vi "Get Map Collection Data Size.vi"(8 "error in (no error)":errorcluster, 10 "Data String":u8[](array[numeric]), 11 "Type Descriptor":i16[](array[numeric])) -> (0 "error out":errorcluster, 2 "Data Size":i32)   [LabVIEW 2017, in "Composition.lvlib"]
doc: "Gets the data size of a map collection."
uses:
  Composition.lvlib
  Get Data Type.vi/2a0888ac-0230-421b-a610-ddb651202d87.vi
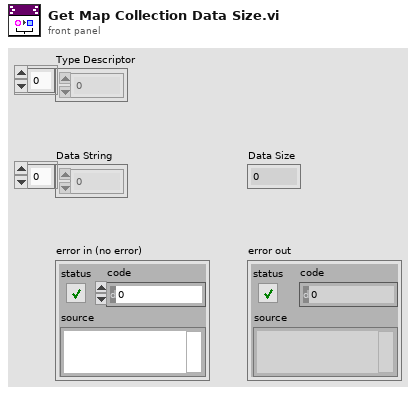
[diagram p1: front panel]
types:
  T1 = typedef "Composition.lvlib/Data Type.ctl" = enum16{"Void", "I8", "I16", "I32", "I64", "U8", "U16", "U32", "U64", "SGL", "DBL", "EXT", "CSG", "CDB", "CXT", "0x0F", "0x10", "0x11", "0x12", "0x13", "0x14", "Enum U8", "Enum U16", "Enum U32", "0x18", "SGL Physical", "DBL Physical", "EXT Physical", "CSG Physical", "CDB Physical", "CXT Physical", "0x1F", "Boolean U16", "Boolean U8", "0x22", "0x23", "0x24", "0x25", "0x26", "0x27", "0x28", "0x29", "0x2A", "0x2B", "0x2C", "0x2D", "0x2E", "0x2F", "String", "0x31", "Path", "Picture", "CString", "PString", "0x36", "Tag", "0x38", "0x39", "0x3A", "0x3B", "0x3C", "0x3D", "0x3E", "SubString", "Array", "Array Data Ptr", "0x42", "0x43", "0x44", "0x45", "0x46", "0x47", "0x48", "0x49", "0x4A", "0x4B", "0x4C", "0x4D", "0x4E", "SubArray", "Cluster", "0x51", "0x52", "Variant", "Waveform", "0x55", "0x56", "0x57", "0x58", "0x59", "0x5A", "0x5B", "0x5C", "0x5D", "CFX", "FXP", "Block", "Type Block", "Void Block", "Aligned Block", "Repeated Block", "Alignment Marker", "0x66", "0x67", "0x68", "0x69", "0x6A", "0x6B", "0x6C", "0x6D", "0x6E", "0x6F", "Refnum", "0x71", "0x72", "Set Collection", "Map Collection", "0x75", "0x76", "0x77", "0x78", "0x79", "0x7A", "0x7B", "0x7C", "0x7D", "0x7E", "0x7F", "Ptr", "0x81", "0x82", "Ptr to", "EXT Data", "0x85", "0x86", "0x87", "0x88", "0x89", "0x8A", "0x8B", "0x8C", "0x8D", "0x8E", "0x8F", "0x90", "0x91", "0x92", "0x93", "0x94", "0x95", "0x96", "0x97", "0x98", "0x99", "0x9A", "0x9B", "0x9C", "0x9D", "0x9E", "0x9F", "Array Interface", "Interface to Data", "0xA2", "0xA3", "0xA4", "0xA5", "0xA6", "0xA7", "0xA8", "0xA9", "0xAA", "0xAB", "0xAC", "0xAD", "0xAE", "0xAF", "0xB0", "0xB1", "0xB2", "0xB3", "0xB4", "0xB5", "0xB6", "0xB7", "0xB8", "0xB9", "0xBA", "0xBB", "0xBC", "0xBD", "0xBE", "0xBF", "0xC0", "0xC1", "0xC2", "0xC3", "0xC4", "0xC5", "0xC6", "0xC7", "0xC8", "0xC9", "0xCA", "0xCB", "0xCC", "0xCD", "0xCE", "0xCF", "0xD0", "0xD1", "0xD2", "0xD3", "0xD4", "0xD5", "0xD6", "0xD7", "0xD8", "0xD9", "0xDA", "0xDB", "0xDC", "0xDD", "0xDE", "0xDF", "0xE0", "0xE1", "0xE2", "0xE3", "0xE4", "0xE5", "0xE6", "0xE7", "0xE8", "0xE9", "0xEA", "0xEB", "0xEC", "0xED", "0xEE", "0xEF", "Function", "TypeDef", "PolyVI", "0xF3", "0xF4", "0xF5", "0xF6", "0xF7", "0xF8", "0xF9", "0xFA", "0xFB", "0xFC", "0xFD", "0xFE", "0xFF"}
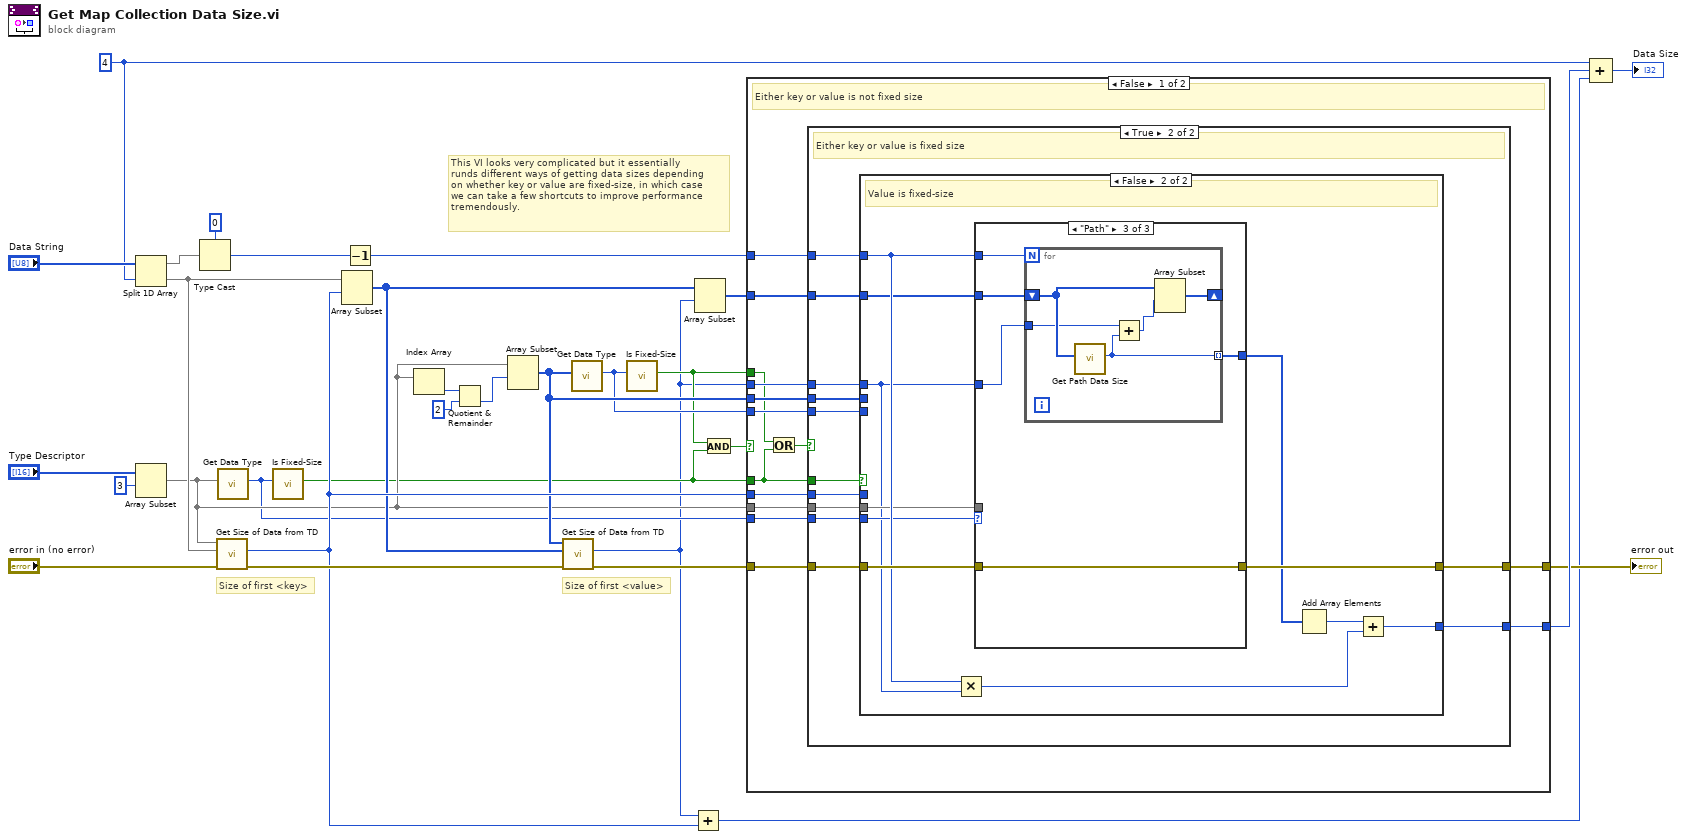
[diagram p0: block diagram]
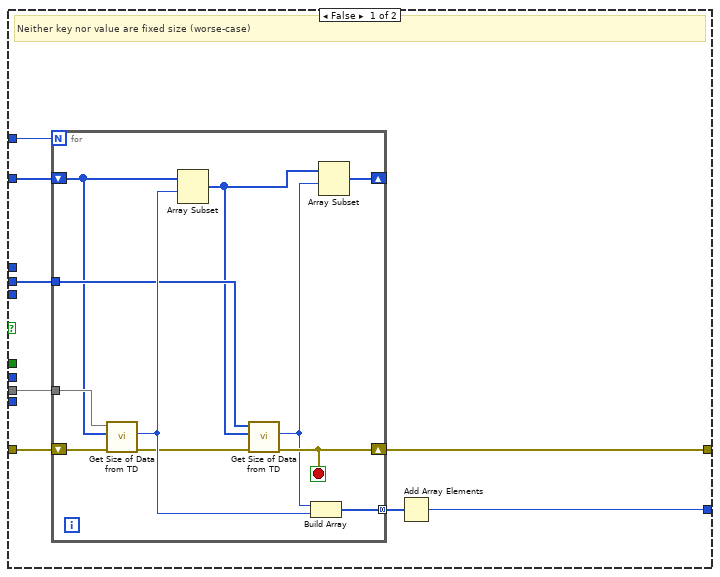
[diagram p2: hidden frame]
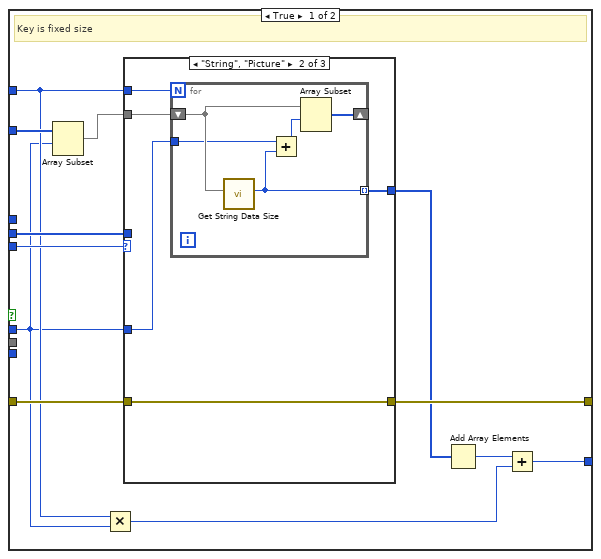
[diagram p3: hidden frame]
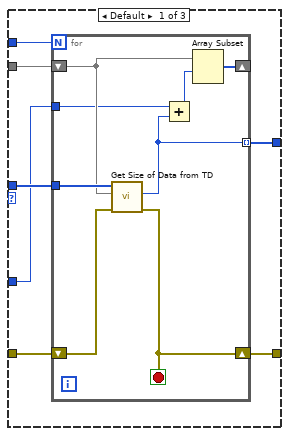
[diagram p4: hidden frame]
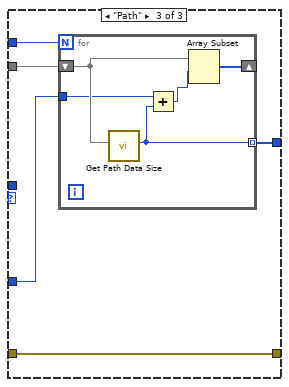
[diagram p5: hidden frame]
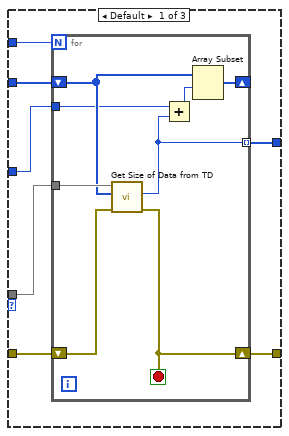
[diagram p6: hidden frame]
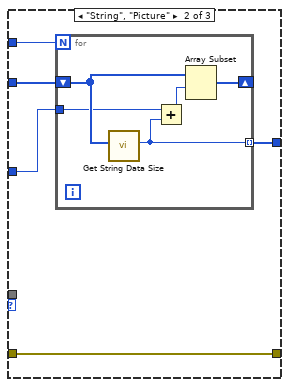
[diagram p7: hidden frame]
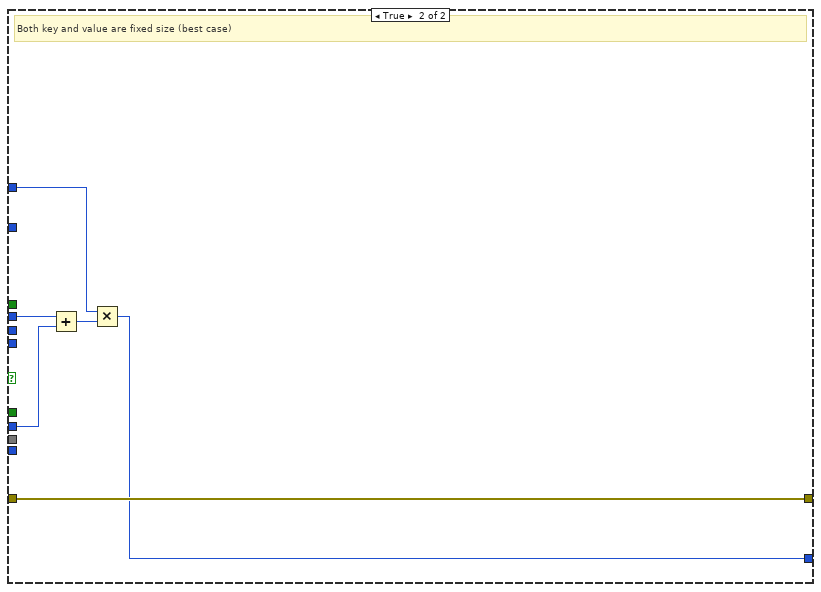
[diagram p8: hidden frame]
diagram:
  w10 = 4 ("index")
  # "This VI looks very complicated but it essentially\nrunds different ways of getting data sizes depending\non whether key or value are fixed-size, in which case\nwe can take a few shortcuts to improve performance\ntremendously."
  # "Size of first <value>"
  # "Size of first <key>"
  n1 = Split 1D Array(array="Data String", index=w10) -> (first subarray=w28:u8[], second subarray=w17:u8[])
  n2 = Array Subset(array="Type Descriptor", index=3) -> (w6:i16[])  [unwired: 1 in]
  n3 = Type Cast(type=0, x=w28) -> (*(type *) &x=w27:i32)
  n4 = call "Get Size of Data from TD.vi"("error in (no error)"="error in (no error)", "Data String"=w17, "Type Descriptor"=w6) -> ("error out"=w16:errorcluster, "Size of Data"=w14:i32)  [unwired: 7 in]
  n5 = call "Get Data Type.vi"("Type Descriptor"=w6) -> ("Data Type"=w5:T1)  [unwired: 10 in]
  n6 = call "Is Fixed-Size.vi"("Data Type"=w5) -> ("Is Fixed-Size"=w2:bool)  [unwired: 10 in]
  n7 = Array Subset(array=w17, index=w14) -> (w9:u8[])  [unwired: 1 in]
  n8 = Decrement(x=w27) -> (x-1=w15:i32)
  n9 = Index Array(array=w6) -> (element=w19:i16)  [unwired: 1 in]
  n10 = Quotient & Remainder(x=w19, y=i16 2) -> (floor(x/y)=w21:i16)  [unwired: 1 out]
  n11 = Array Subset(array=w6, index=w21) -> (w12:i16[])  [unwired: 1 in]
  n12 = call "Get Size of Data from TD.vi"("error in (no error)"=w16, "Data String"=w9, "Type Descriptor"=w12) -> ("error out"=w11:errorcluster, "Size of Data"=w1:i32)  [unwired: 7 in]
  n13 = call "Get Data Type.vi"("Type Descriptor"=w12) -> ("Data Type"=w7:T1)  [unwired: 10 in]
  n14 = call "Is Fixed-Size.vi"("Data Type"=w7) -> ("Is Fixed-Size"=w3:bool)  [unwired: 10 in]
  n15 = Add(x=w1, y=w14) -> (x+y=w13:i32)
  n16 = Array Subset(array=w9, index=w1) -> (w8:u8[])  [unwired: 1 in]
  n17 = And(x=w3, y=w2) -> (x .and. y?=w4:bool)
  n18 = case shown="False" w4 {
    tunnel: [w44 w169] -> w26
    tunnel: [w43 w174] -> w23
    tunnel: w15 -> [w42 w170]
    tunnel: w2 -> [w33 _]
    tunnel: w3 -> [w32 _]
    tunnel: w14 -> [w41 w172]
    tunnel: w12 -> [w40 _]
    tunnel: w11 -> [w39 w174]
    tunnel: w8 -> [w38 _]
    tunnel: w1 -> [w37 w173]
    tunnel: w7 -> [w36 _]
    tunnel: w6 -> [w35 _]
    tunnel: w5 -> [w34 _]
    frame False {
      # "Either key or value is not fixed size"
      n19 = Or(x=w32, y=w33) -> (x .or. y?=w31:bool)
      n20 = case shown="True" w31 {
        tunnel: [w51 w67] -> w44
        tunnel: [w50 w75] -> w43
        tunnel: w42 -> [w49 w74]
        tunnel: w33 -> [_ w69]
        tunnel: w41 -> [_ w68]
        tunnel: w40 -> [w48 w73]
        tunnel: w39 -> [w47 w72]
        tunnel: w38 -> [w46 w71]
        tunnel: w37 -> [_ w66]
        tunnel: w36 -> [_ w65]
        tunnel: w35 -> [w45 w70]
        tunnel: w34 -> [_ w64]
        frame False {
          # "Neither key nor value are fixed size (worse-case)"
          n21 = for {
            N: w49 -> [_]
            shift-right: [w63] -> _
            shift-left: w46 -> [w53]
            tunnel: [w61] -> w52 mode=concatenating
            shift-right: [w59] -> w50
            shift-left: w47 -> [w60]
            tunnel: w45 -> [w56]
            tunnel: w48 -> [w55]
            stop <- w59 stop-if-true
            n22 = call "Get Size of Data from TD.vi"("error in (no error)"=w60, "Data String"=w53, "Type Descriptor"=w56) -> ("error out"=w57:errorcluster, "Size of Data"=w62:i32)  [unwired: 7 in]
            n23 = Array Subset(array=w53, index=w62) -> (w54:u8[])  [unwired: 1 in]
            n24 = call "Get Size of Data from TD.vi"("error in (no error)"=w57, "Data String"=w54, "Type Descriptor"=w55) -> ("error out"=w59:errorcluster, "Size of Data"=w58:i32)  [unwired: 7 in]
            n25 = Build Array(w58, w62) -> (w61:i32[])
            n26 = Array Subset(array=w54, index=w58) -> (w63:u8[])  [unwired: 1 in]
          }
          n27 = Add Array Elements(numeric array=w52) -> (sum=w51:i32)
        }
        frame True {
          # "Either key or value is fixed size"
          n28 = case shown="False" w69 {
            tunnel: [w85 w132] -> w67
            tunnel: [w83 w130] -> w75
            tunnel: w74 -> [w79 w128]
            tunnel: w73 -> [w81 _]
            tunnel: w72 -> [w82 w129]
            tunnel: w71 -> [w87 w123]
            tunnel: w70 -> [_ w126]
            tunnel: w68 -> [w76 _]
            tunnel: w66 -> [_ w124]
            tunnel: w65 -> [w80 _]
            tunnel: w64 -> [_ w125]
            frame True {
              # "Key is fixed size"
              n29 = Array Subset(array=w87, index=w76) -> (w78:u8[])  [unwired: 1 in]
              n30 = Multiply(x=w79, y=w76) -> (x*y=w84:i32)
              n31 = case shown="\"String\", \"Picture\"" w80 {
                tunnel: w78 -> [w94 w106 w116]
                tunnel: w79 -> [w93 w107 w117]
                tunnel: [w89 w104 w114] -> w77
                tunnel: w81 -> [w92 _ _]
                tunnel: w82 -> [w91 w105 w115]
                tunnel: [w90 w105 w115] -> w83
                tunnel: w76 -> [w88 w103 w113]
                frame Default {
                  n32 = for {
                    N: w93 -> [_]
                    tunnel: w92 -> [w102]
                    shift-right: [w100] -> _
                    shift-left: w94 -> [w101]
                    tunnel: [w97] -> w89 mode=indexing
                    shift-right: [w98] -> w90
                    shift-left: w91 -> [w99]
                    tunnel: w88 -> [w96]
                    stop <- w98 stop-if-true
                    n33 = call "Get Size of Data from TD.vi"("error in (no error)"=w99, "Data String"=w101, "Type Descriptor"=w102) -> ("error out"=w98:errorcluster, "Size of Data"=w97:i32)  [unwired: 7 in]
                    n34 = Add(x=w96, y=w97) -> (x+y=w95:i32)
                    n35 = Array Subset(array=w101, index=w95) -> (w100:u8[])  [unwired: 1 in]
                  }
                }
                frame "String", "Picture" {
                  n36 = for {
                    N: w107 -> [_]
                    shift-right: [w112] -> _
                    shift-left: w106 -> [w111]
                    tunnel: [w110] -> w104 mode=indexing
                    tunnel: w103 -> [w108]
                    n37 = call "Get String Data Size.vi"("Data String"=w111) -> ("Data Size"=w110:i32)  [unwired: 10 in]
                    n38 = Add(x=w108, y=w110) -> (x+y=w109:i32)
                    n39 = Array Subset(array=w111, index=w109) -> (w112:u8[])  [unwired: 1 in]
                  }
                }
                frame "Path" {
                  n40 = for {
                    N: w117 -> [_]
                    shift-right: [w122] -> _
                    shift-left: w116 -> [w121]
                    tunnel: [w120] -> w114 mode=indexing
                    tunnel: w113 -> [w118]
                    n41 = call "Get Path Data Size.vi"("Data String"=w121) -> ("Data Size"=w120:i32)  [unwired: 10 in]
                    n42 = Add(x=w118, y=w120) -> (x+y=w119:i32)
                    n43 = Array Subset(array=w121, index=w119) -> (w122:u8[])  [unwired: 1 in]
                  }
                }
              }
              n44 = Add Array Elements(numeric array=w77) -> (sum=w86:i32)
              n45 = Add(x=w86, y=w84) -> (x+y=w85:i32)
            }
            frame False {
              # "Value is fixed-size"
              n46 = Multiply(x=w128, y=w124) -> (x*y=w131:i32)
              n47 = case shown="\"Path\"" w125 {
                tunnel: w123 -> [w140 w152 w162]
                tunnel: w128 -> [w139 w153 w163]
                tunnel: [w135 w150 w160] -> w127
                tunnel: w126 -> [w138 _ _]
                tunnel: w129 -> [w137 w151 w161]
                tunnel: [w136 w151 w161] -> w130
                tunnel: w124 -> [w134 w149 w159]
                frame Default {
                  n48 = for {
                    N: w139 -> [_]
                    tunnel: w138 -> [w148]
                    shift-right: [w146] -> _
                    shift-left: w140 -> [w147]
                    tunnel: [w143] -> w135 mode=indexing
                    shift-right: [w144] -> w136
                    shift-left: w137 -> [w145]
                    tunnel: w134 -> [w142]
                    stop <- w144 stop-if-true
                    n49 = call "Get Size of Data from TD.vi"("error in (no error)"=w145, "Data String"=w147, "Type Descriptor"=w148) -> ("error out"=w144:errorcluster, "Size of Data"=w143:i32)  [unwired: 7 in]
                    n50 = Add(x=w142, y=w143) -> (x+y=w141:i32)
                    n51 = Array Subset(array=w147, index=w141) -> (w146:u8[])  [unwired: 1 in]
                  }
                }
                frame "String", "Picture" {
                  n52 = for {
                    N: w153 -> [_]
                    shift-right: [w158] -> _
                    shift-left: w152 -> [w157]
                    tunnel: [w156] -> w150 mode=indexing
                    tunnel: w149 -> [w154]
                    n53 = call "Get String Data Size.vi"("Data String"=w157) -> ("Data Size"=w156:i32)  [unwired: 10 in]
                    n54 = Add(x=w154, y=w156) -> (x+y=w155:i32)
                    n55 = Array Subset(array=w157, index=w155) -> (w158:u8[])  [unwired: 1 in]
                  }
                }
                frame "Path" {
                  n56 = for {
                    N: w163 -> [_]
                    shift-right: [w168] -> _
                    shift-left: w162 -> [w167]
                    tunnel: [w166] -> w160 mode=indexing
                    tunnel: w159 -> [w164]
                    n57 = call "Get Path Data Size.vi"("Data String"=w167) -> ("Data Size"=w166:i32)  [unwired: 10 in]
                    n58 = Add(x=w164, y=w166) -> (x+y=w165:i32)
                    n59 = Array Subset(array=w167, index=w165) -> (w168:u8[])  [unwired: 1 in]
                  }
                }
              }
              n60 = Add Array Elements(numeric array=w127) -> (sum=w133:i32)
              n61 = Add(x=w133, y=w131) -> (x+y=w132:i32)
            }
          }
        }
      }
    }
    frame True {
      # "Both key and value are fixed size (best case)"
      n62 = Add(x=w173, y=w172) -> (x+y=w171:i32)
      n63 = Multiply(x=w170, y=w171) -> (x*y=w169:i32)
    }
  }
  "error out" <- w23
  n64 = Compound Arithmetic op=ADD(w10, w26, w13) -> (→"Data Size":i32)
